vi "Remove test suites.vi"(6 "Linker.Read Info From File":T2(array[cluster]), 9 "Define Test index":i32, 10 "Define Test Suite index":i32, 11 "Directory to search":path) -> (3 "Tests":path[](array[path]))   [LabVIEW 2020, in "Caraya.lvlib" / "Test Runner.Folder.lvclass"]
uses:
  Test Runner.Folder.lvclass
  <vilib>/Utility/lvfile.llb/LVFileType.ctl
  <vilib>/Utility/lvfile.llb/NI_FileType.lvlib
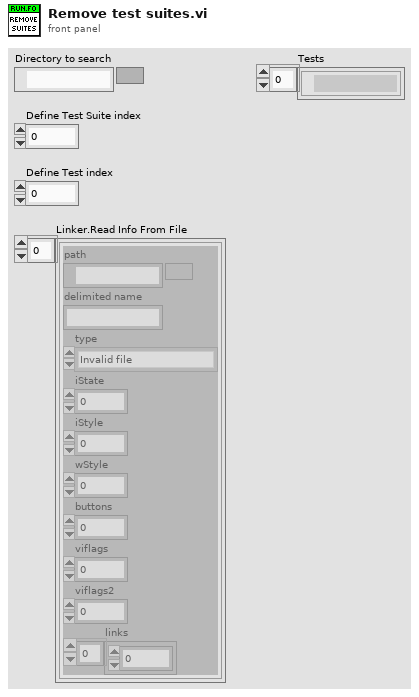
[diagram p1: front panel]
types:
  T1 = typedef "NI_FileType.lvlib/LVFileType.ctl" = enum32{"Invalid file", "Unknown type", "Instrument", "Control", "Polymorphic VI", "Project", "Library", "LVClass", "XControl", "XNode", "Shared library", ".NET assembly", "ActiveX interface", "CIN", "Run-time menu", "Palette menu", "Help file", "LLB", "XNode Edit Dependency", "Class Private Data Control", "Statechart", "MathScript .m file", "Ladder Diagram", "LVLibp", "XNode Build Dependency"}
  T2 = cluster{"path":path, "delimited name":string, "type":T1, "iState":u32, "iStyle":u16, "wStyle":u16, "buttons":u16, "viflags":u32, "viflags2":u32, "links":u32[]}[]
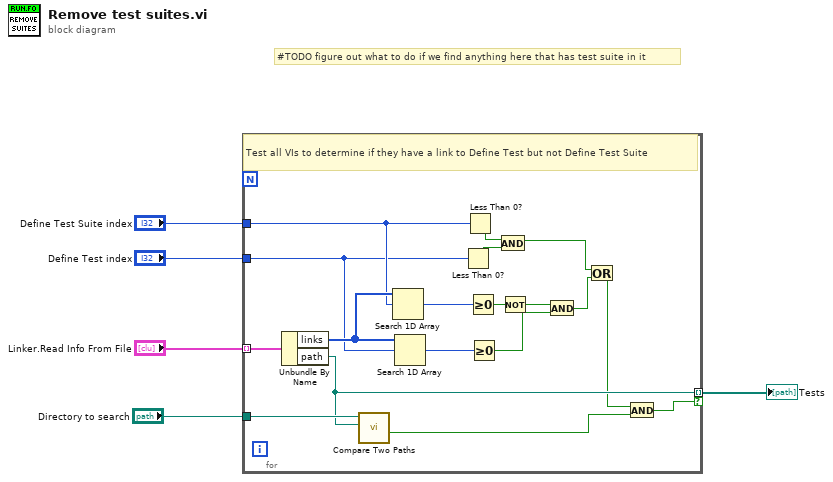
[diagram p0: block diagram]
diagram:
  # "#TODO figure out what to do if we find anything here that has test suite in it"
  n1 = for {
    tunnel: "Linker.Read Info From File" -> [w23] mode=indexing
    tunnel: "Define Test Suite index" -> [w12]
    tunnel: "Define Test index" -> [w11]
    tunnel: [w15] -> w5 mode=indexing if=w14
    tunnel: "Directory to search" -> [w16]
    # "Test all VIs to determine if they have a link to Define Test but not Define Test Suite"
    n2 = Unbundle By Name(w23) -> ("links"=w22:u32[], "path"=w15:path)
    n3 = call <vilib>:"Compare Two Paths.vi"("Path 2"=w15, "Path 1"=w16) -> ("Path 2 Relative to Path 1?"=w13:bool)  [unwired: 6 in, 3 out]
    n4 = Search 1D Array(1D array=w22, element=w12) -> (index of element=w21:i32)  [unwired: 1 in]
    n5 = Search 1D Array(1D array=w22, element=w11) -> (index of element=w20:i32)  [unwired: 1 in]
    n6 = Less Than 0?(x=w11) -> (x < 0?=w10:bool)
    n7 = Less Than 0?(x=w12) -> (x < 0?=w9:bool)
    n8 = Greater Or Equal To 0?(x=w21) -> (x >= 0?=w18:bool)
    n9 = Greater Or Equal To 0?(x=w20) -> (x >= 0?=w19:bool)
    n10 = And(x=w9, y=w10) -> (x .and. y?=w8:bool)
    n11 = Not(x=w18) -> (.not. x?=w17:bool)
    n12 = And(x=w17, y=w19) -> (x .and. y?=w7:bool)
    n13 = Or(x=w8, y=w7) -> (x .or. y?=w6:bool)
    n14 = And(x=w6, y=w13) -> (x .and. y?=w14:bool)
  }
  "Tests" <- w5
